vi "New.vi"(11 "age limit [days](30)":dbl=30.0) -> (3 "Cleanup Filter":refnum<class "CleanupFilter.LastMod.lvclass">)   [LabVIEW 2018, in "GLog.lvlib" / "CleanupFilter.LastMod.lvclass"]
uses:
  CleanupFilter.LastMod.lvclass
  CleanupFilter.LastMod.lvclass/CleanupFilter.LastMod.ctl
panel:
  # "Connector Pane"
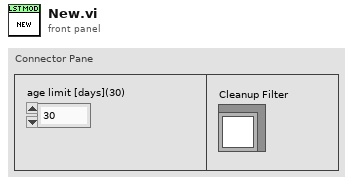
[diagram p1: front panel]
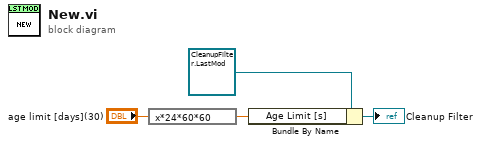
[diagram p0: block diagram]
diagram:
  n1 = expression code="x*24*60*60"("age limit [days](30)") -> (w1:dbl)
  n2 = Bundle By Name(cluster=refnum<class "CleanupFilter.LastMod.lvclass"> refnum ("CleanupFilter.LastMod in"), "Age Limit [s]"=w1) -> (→"Cleanup Filter":refnum<class "CleanupFilter.LastMod.lvclass">)
